vi "RemoteVI Share Running.vi"(0 "port":u16=8088) -> (4 "running?":bool)   [LabVIEW 2020, in "RemoteVI.lvlib"]
doc: "TRUE when a RemoteVI share of this LabVIEW application instance serves port right now - its server loop published its status within the last 2 s (RemoteVI Status Registry.vi, RemoteVI Status Convert.vi). Used by RemoteVI Start.vi, which then launches nothing (error 5001); a share whose loop was aborted is no longer running after 2 s."
uses:
  RemoteVI.lvlib
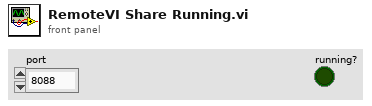
[diagram p1: front panel]
types:
  T1 = cluster{"port":u16, "url":string, "target":string, "kind":string, "whole network":bool, "started":dbl, "updated":dbl, "clients":cluster{"address":string, "since":dbl, "last input":dbl}[], "fps":dbl, "bytes per s":dbl, "frames":u32, "latency ms":dbl, "view only":bool, "last error":string, "hWnd":u64}[]
  T2 = cluster{"port":u16, "url":string, "target":string, "kind":string, "whole network":bool, "running":bool, "uptime s":dbl, "clients":cluster{"address":string, "connected s":dbl, "idle s":dbl}[], "fps":dbl, "kB per s":dbl, "frames":u32, "latency ms":dbl, "view only":bool, "last error":string, "hWnd":u64}[]
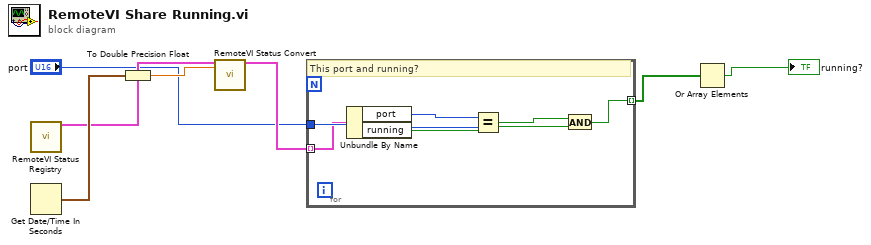
[diagram p0: block diagram]
diagram:
  n1 = call "RemoteVI Status Registry.vi"() -> ("servers"=w2:T1)  [unwired: 15 in]
  n2 = Get Date/Time In Seconds() -> (seconds since 1Jan1904=w3:timestamp)
  n3 = To Double Precision Float(number=w3) -> (double precision float=w4:dbl)
  n4 = call "RemoteVI Status Convert.vi"("raw"=w2, "now"=w4) -> ("status"=w5:T2)  [unwired: 13 in]
  n5 = for {
    tunnel: "port" -> [w9]
    tunnel: w5 -> [w8] mode=indexing
    tunnel: [w13] -> w6 mode=indexing
    # "This port and running?"
    n6 = Unbundle By Name(w8) -> ("port"=w10:u16, "running"=w11:bool)
    n7 = Equal?(x=w10, y=w9) -> (x = y?=w12:bool)
    n8 = And(x=w12, y=w11) -> (x .and. y?=w13:bool)
  }
  n9 = Or Array Elements(Boolean array=w6) -> (logical OR=→"running?":bool)
